vi "VIH Project Tree - Find Invalid Files in Project Tree.vi"(8 "error in":errorcluster, 11 "Project Tree":T1) -> (0 "error out":errorcluster, 1 "Item Paths":path[](array[path]), 2 "Tree Item Tags":string[](array[string]), 3 "dup Project Tree":T1)   [LabVIEW 2014]
doc: "::: VI Helpeks :::\nCopyright (c) 2000-2026 Konstantin Shifershteyn. All rights reserved."
uses:
  VIH Project Tree Typedef - Tree Refnum.ctl
panel:
  # "VI Helpeks\nCopyright (c) 2012-2026 Konstantin Shifershteyn"
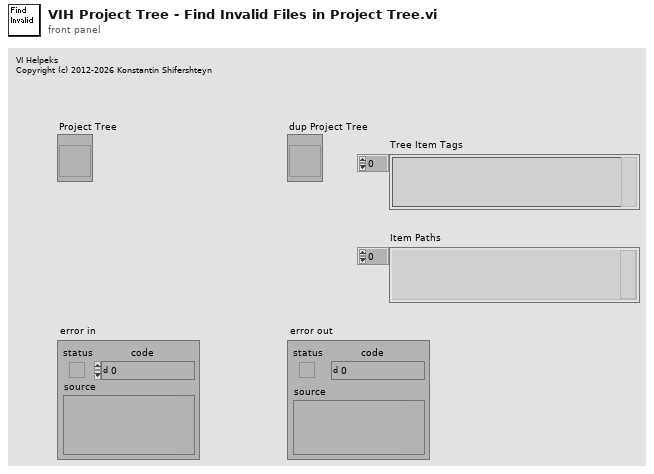
[diagram p1: front panel]
types:
  T1 = typedef "VIH Project Tree Typedef - Tree Refnum.ctl" = refnum<vi>
  T2 = typedef "VIH Project Tree Typedef - Tree Item Type.ctl" = enum32{"<Invalid>", "Project", "Proj Files", "Proj Rules", "File Group", "Rule Group", "Any File", "LV Func", ".mnu", ".mnu (dyn)", ".vi", ".vi (dyn)", ".vit", ".vit (dyn)", ".ctl", ".ctl (dyn)", ".ctt", ".ctt (dyn)", "polyVI", "polyVI (dyn)", "expVI", "expVI (dyn)", "HTML", "PolyVI Inst"}
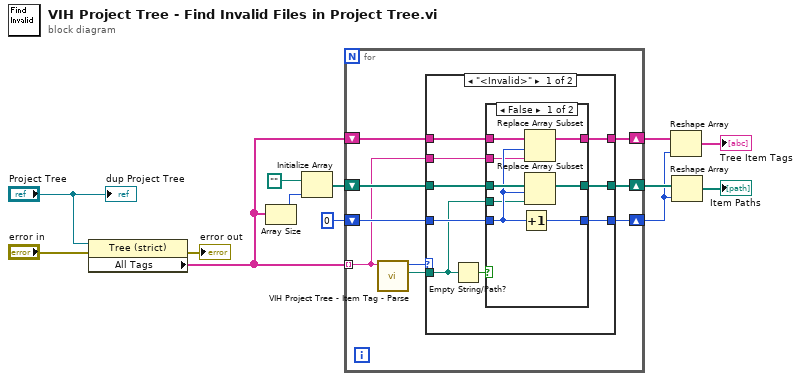
[diagram p0: block diagram]
diagram:
  n1 = property on="Property Node" class="Tree (strict)"(reference="Project Tree", error in="error in") -> (error out=→"error out":errorcluster, "All Tags"=w6:string[])  [unwired: 1 out]
  n2 = Array Size(array=w6) -> (size(s)=w9:i32)
  n3 = Initialize Array(path "", w9) -> (w8:path[])
  n4 = for {
    tunnel: w6 -> [w14] mode=indexing
    shift-right: [w20] -> w5
    shift-left: w6 -> [w21]
    shift-right: [w18] -> w4
    shift-left: w8 -> [w19]
    shift-right: [w16] -> w3
    shift-left: 0 -> [w17]
    n5 = call "VIH Project Tree - Item Tag - Parse.vi"("Tree Item Tag"=w14) -> ("Item File Path"=w15:path, "Item Type"=w22:T2)  [unwired: 8 in, 1 out]
    n6 = case shown="\"<Invalid>\"" w22 {
      tunnel: w21 -> [w29 w45]
      tunnel: [w30 w45] -> w20
      tunnel: w19 -> [w27 w44]
      tunnel: [w28 w44] -> w18
      tunnel: w17 -> [w25 w43]
      tunnel: [w26 w43] -> w16
      tunnel: w15 -> [w24 _]
      tunnel: w14 -> [w23 _]
      frame "<Invalid>" {
        n7 = Empty String/Path?(string/path=w24) -> (empty?=w31:bool)
        n8 = case shown="False" w31 {
          tunnel: [w38 w42] -> w30
          tunnel: w29 -> [w39 w42]
          tunnel: [w36 w41] -> w28
          tunnel: w27 -> [w37 w41]
          tunnel: [w35 w40] -> w26
          tunnel: w25 -> [w34 w40]
          tunnel: w24 -> [w33 _]
          tunnel: w23 -> [w32 _]
          frame False {
            n9 = Increment(x=w34) -> (x+1=w35:i32)
            n10 = Replace Array Subset(array=w39, new element=w32, index=w34) -> (w38:string[])
            n11 = Replace Array Subset(array=w37, new element=w33, index=w34) -> (w36:path[])
          }
          frame True {
          }
        }
      }
      frame Default {
      }
    }
  }
  n12 = Reshape Array(w5, w3) -> (→"Tree Item Tags":string[])
  n13 = Reshape Array(w4, w3) -> (→"Item Paths":path[])
  "dup Project Tree" <- "Project Tree"
